vi "Progress_Bar.vi"(8 "error out":errorcluster, 10 "stop":bool) -> (0 "error out":errorcluster)   [LabVIEW 2021]
panel:
  out "Slide":u8(slide) scale=0.0..100.0
  # "INITIALIZING INSTRUMENT"
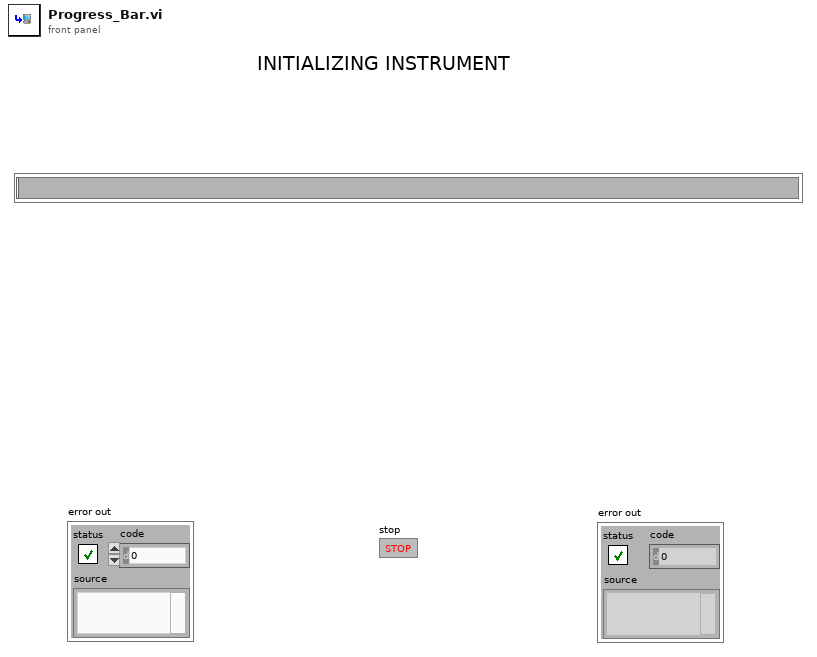
[diagram p1: front panel]
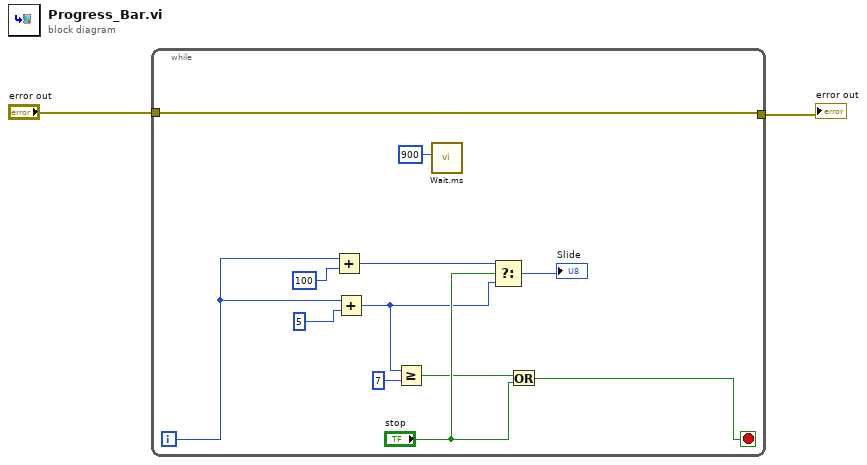
[diagram p0: block diagram]
diagram:
  n1 = while {
    tunnel: "error out" -> [w3]
    tunnel: [w3] -> w1
    i -> [w8]
    stop <- w4 stop-if-true
    n2 = Add(x=w8, y=100) -> (x+y=w11:i32)
    n3 = Add(x=w8, y=5) -> (x+y=w5:i32)
    n4 = Greater Or Equal?(x=w5, y=7) -> (x >= y?=w6:bool)
    n5 = call "Wait.ms.vi"("milliseconds to wait"=u32 900) -> ()  [unwired: 10 in, 1 out]
    n6 = Select(t=w11, s="stop", f=w5) -> (s? t:f=→"Slide":i32)
    n7 = Or(x=w6, y="stop") -> (x .or. y?=w4:bool)
  }
  "error out" <- w1
